vi "Read Collection.vi"(11 "Test Runner.Collection in":refnum<class "Test Runner.Collection.lvclass">) -> (2 "Test Runners":refnum<class "Test Runner.lvclass">[](array[class]), 3 "Test Runner.Collection out":refnum<class "Test Runner.Collection.lvclass">)   [LabVIEW 2020, in "Caraya.lvlib" / "Test Runner.Collection.lvclass"]
uses:
  Test Runner.Collection.lvclass
  Test Runner/Test Runner.lvclass
  Test Runner.Collection.lvclass/Test Runner.Collection.ctl
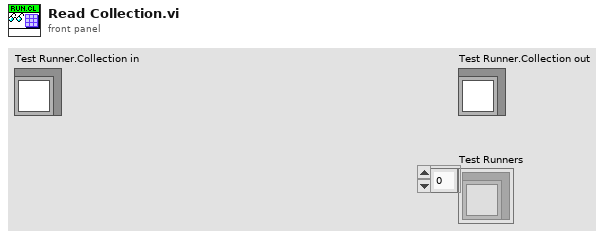
[diagram p1: front panel]
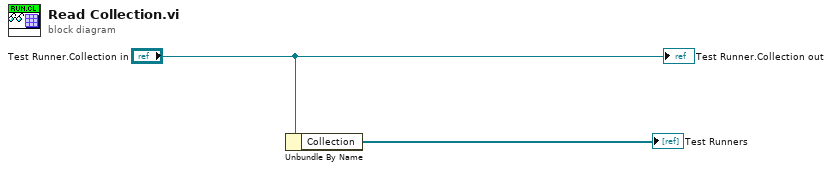
[diagram p0: block diagram]
diagram:
  n1 = Unbundle By Name("Test Runner.Collection in") -> ("Collection"=→"Test Runners":refnum<class "Test Runner.lvclass">[])
  "Test Runner.Collection out" <- "Test Runner.Collection in"
